vi "Main.vi"   [LabVIEW 2022 SP3]
uses:
  <vilib>/addons/Qbus/Qbus.lvclass
  processes/ManageConnection/AudioGenManageConnectionProcess.lvlib
  shared/logger process/EventLoggerProcess.lvlib
  <vilib>/addons/PointValueMap/PointValueMap.lvlib
  processes/TCP Read/AudioGenTCPReaderProcess.lvlib
  processes/Digital Audio Generation/DigitalAudioGenerationProcess.lvlib
  subVIs/utility/AudioGenUtility.lvlib
  processes/Analog Generation/AnalogGenerationProcess.lvlib
types:
  T1 = enum32{"Invalid", "Standard", "Closed", "Hidden", "Minimized", "Maximized"}
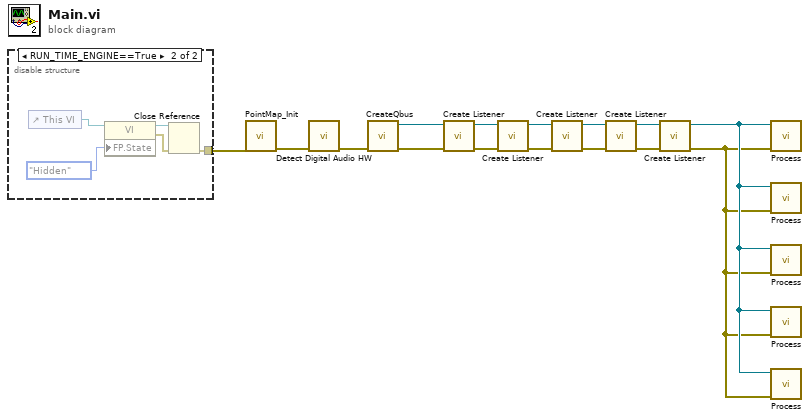
[diagram p0: block diagram]
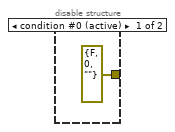
[diagram p2: hidden frame]
diagram:
  n1 = disable-structure shown="RUN_TIME_ENGINE==True" {
    disable-tunnel: [errorcluster {"status"=FALSE, "code"=0, "source"=""} ("error in (no error)") w17] -> w5
    frame condition #0 (active) {
    }
    frame condition #1 {
      n2 = control-ref of="This VI"() -> (w20:refnum<vi>)
      n3 = property class="VI"(reference=w20, "FP.State"=T1."Hidden" ("Front Panel Window:State")) -> (reference out=w19:refnum<vi>, error out=w18:errorcluster)  [unwired: 1 in]
      n4 = Close Reference(reference=w19, error in (no error)=w18) -> (error out=w17:errorcluster)
    }
  }
  n5 = call <vilib>:"PointMap_Init.vi"("error in (no error)"=w5) -> ("error out"=w7:errorcluster)  [unwired: 10 in]
  n6 = call "Detect Digital Audio HW.vi"("error in (no error)"=w7) -> ("error out"=w6:errorcluster)  [unwired: 9 in, 1 out]
  n7 = call <vilib>:"CreateQbus.vi"("error in (no error)"=w6) -> ("error out"=w14:errorcluster, "Qbus"=w15:refnum<class "Qbus.lvclass">)  [unwired: 9 in]
  n8 = call "Create Listener.vi"("error in (no error)"=w14, "Qbus in"=w15) -> ("error out"=w13:errorcluster, "Qbus out"=w12:refnum<class "Qbus.lvclass">)  [unwired: 8 in]
  n9 = call "Create Listener.vi"("error in (no error)"=w13, "Qbus in"=w12) -> ("error out"=w10:errorcluster, "Qbus out"=w11:refnum<class "Qbus.lvclass">)  [unwired: 8 in]
  n10 = call "Create Listener.vi"("error in (no error)"=w10, "Qbus in"=w11) -> ("error out"=w8:errorcluster, "Qbus out"=w9:refnum<class "Qbus.lvclass">)  [unwired: 8 in]
  n11 = call "Create Listener.vi"("error in (no error)"=w8, "Qbus in"=w9) -> ("error out"=w4:errorcluster, "Qbus out"=w3:refnum<class "Qbus.lvclass">)  [unwired: 8 in]
  n12 = call "Create Listener.vi"("error in (no error)"=w4, "Qbus in"=w3) -> ("error out"=w1:errorcluster, "Qbus out"=w2:refnum<class "Qbus.lvclass">)  [unwired: 8 in]
  n13 = call "Process.vi"("error in"=w1, "Qbus in"=w2) -> ()  [unwired: 9 in, 1 out]
  n14 = call "Process.vi"("error in"=w1, "Qbus in"=w2) -> ()  [unwired: 9 in, 1 out]
  n15 = call "Process.vi"("error in"=w1, "Qbus in"=w2) -> ()  [unwired: 9 in, 1 out]
  n16 = call "Process.vi"("error in"=w1, "Qbus in"=w2) -> ()  [unwired: 9 in, 1 out]
  n17 = call "Process.vi"("error in"=w1, "Qbus in"=w2) -> ()  [unwired: 9 in, 1 out]
